vi "Global Language Selection.vi"() -> ()   [LabVIEW 2019, in "Language Selection.lvlib"]
doc: "- - -\nCopyright (c) 2026, Merecs Engineering GmbH"
uses:
  Language Selection.lvlib
  Cluster DVR.ctl
  community/Cluster Settings Data.ctl
  TypeDefs/Cluster LanguageClusterWithRefnum.ctl
  TypeDefs/Cluster PropertyTranslation.ctl
  TypeDefs/Enum Property Type.ctl
panel:
  in  "Translation file path":path
  out "DVR":refnum<data-value>
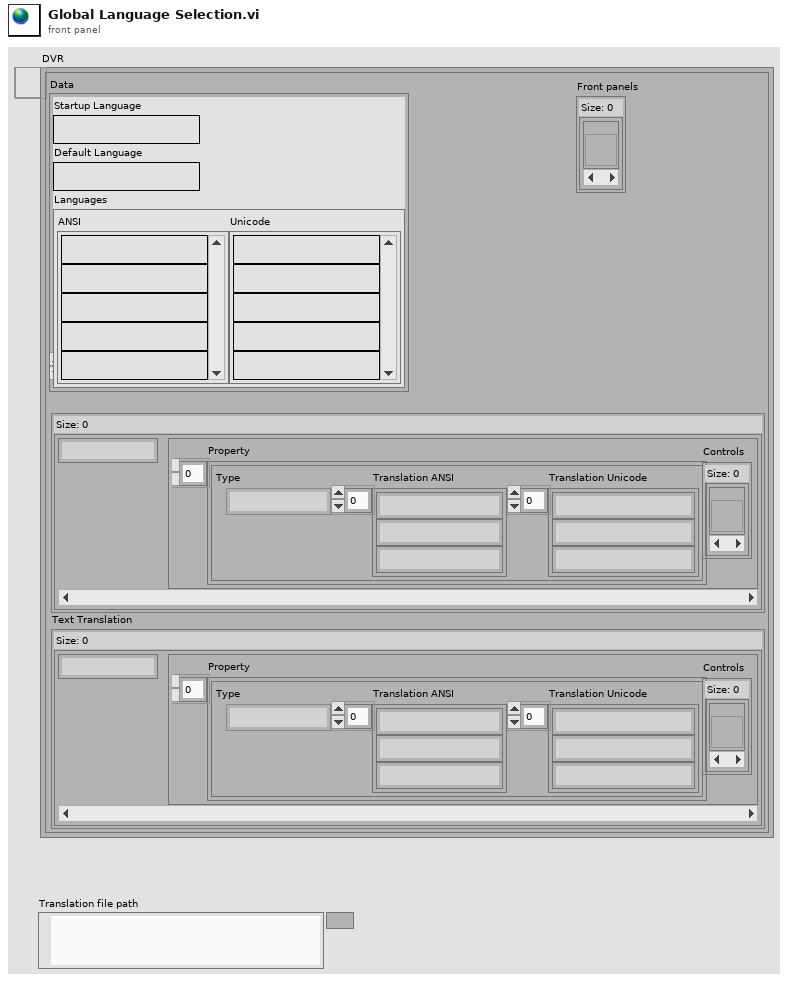
[diagram p1: front panel]
diagram:
